vi "Measurement Logic.vi"() -> ()   [LabVIEW 2021, in "Efficiency And Load Regulation_PMIC.lvlib"]
uses:
  Efficiency And Load Regulation_PMIC.lvlib
  Measurement Configuration.ctl
  Measurement Results.ctl
  <vilib>/Plug-In SDKs/Measurements/Measure Call Context/Measure Call Context.lvclass
  <instrlib>/niDCPower/nidcpower.llb/niDCPower Sense.ctl
  <instrlib>/niDCPower/nidcpower.llb/niDCPower Source Mode.ctl
  <instrlib>/niDCPower/nidcpower.llb/niDCPower Wait For Event - Event.ctl
  <instrlib>/niDCPower/nidcpower.llb/niDCPower Output Function.ctl
  <instrlib>/niDCPower/nidcpower.llb/niDCPower Sequence Attribute Type.ctl
  <instrlib>/niDCPower/nidcpower.llb/niDCPower Get Channel Name From String.vi
  <instrlib>/niDCPower/nidcpower.llb/niDCPower Create Advanced Sequence Step With Channels.vi
  <instrlib>/niDCPower/nidcpower.llb/niDCPower Configure Digital Edge Source Trigger With Channels.vi
  <instrlib>/niDCPower/nidcpower.llb/niDCPower Configure Digital Edge Measure Trigger With Channels.vi
panel:
  out "measure call context out":refnum<class "Measure Call Context.lvclass">
  in  "measure call context in":refnum<class "Measure Call Context.lvclass">
  out "measurement results":T1
  in  "measurement configuration":T2={"Mode of operation"=enum."Perform measurement", "DUT setup time"=1.0, "Source delay"=0.005, "Aperture time"=0.005, "Nominal output voltage"=3.3, "Measurement timeout"=10.0, "Source resource name"="", "Source sense"=1009, "Source current limit"=25.0, "Source maximum power"=300.0, "Source start voltage"=5.0, "Source stop voltage"=20.0, "Source voltage sweep points"=10, "Load resource name"="", "Load sense"=1009, "Load voltage limit range"=6.0, "Load sweep type"="Logarithmic", "Load start current"=0.1, "Load stop current"=24.0, "Load current sweep points/points per decade"=10} {"Load sense" items=["Local"=1008, "Remote"=1009]; "Source sense" items=["Local"=1008, "Remote"=1009]}
  out "error out":errorcluster
  in  "error in":errorcluster
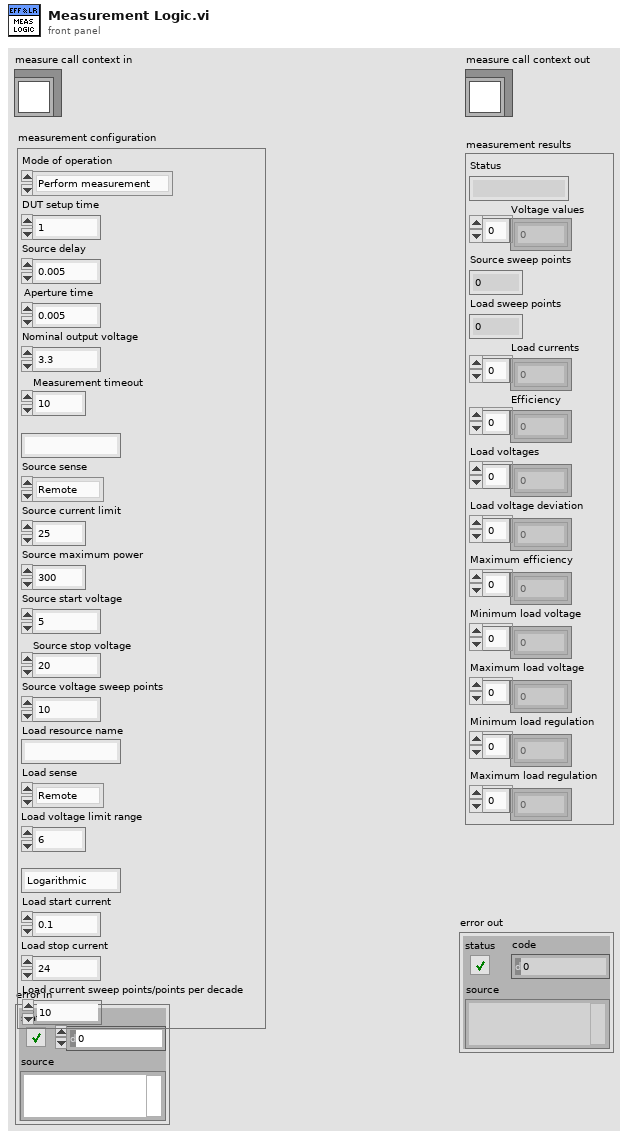
[diagram p1: front panel]
types:
  T1 = typedef "Efficiency And Load Regulation_PMIC.lvlib/Measurement Results.ctl" = cluster{"Status":string, "Voltage values":dbl[], "Source sweep points":i32, "Load sweep points":i32, "Load currents":dbl[], "Efficiency":dbl[], "Load voltages":dbl[], "Load voltage deviation":dbl[], "Maximum efficiency":dbl[], "Minimum load voltage":dbl[], "Maximum load voltage":dbl[], "Minimum load regulation":dbl[], "Maximum load regulation":dbl[]}
  T2 = typedef "Efficiency And Load Regulation_PMIC.lvlib/Measurement Configuration.ctl" = cluster{"Mode of operation":enum32{"Power on the DUT", "Perform measurement", "Power off the DUT"}, "DUT setup time":dbl, "Source delay":dbl, "Aperture time":dbl, "Nominal output voltage":dbl, "Measurement timeout":dbl, "Source resource name":string, "Source sense":i32, "Source current limit":dbl, "Source maximum power":dbl, "Source start voltage":dbl, "Source stop voltage":dbl, "Source voltage sweep points":i32, "Load resource name":string, "Load sense":i32, "Load voltage limit range":dbl, "Load sweep type":string, "Load start current":dbl, "Load stop current":dbl, "Load current sweep points/points per decade":i32}
  T3 = cluster{"Voltage values":dbl[], "Source out":refnum<k15>, "Source channel name":string, "Load out":refnum<k15>, "Load channel name":string, "Current values":dbl[], "Load sweep points":i32, "Source terminal name":string, "Measure terminal name":string, "Measurement Results":T1, "Source sequence name":string}
  T4 = enum32{"Power on the DUT", "Perform measurement", "Power off the DUT"}
  T5 = typedef "niDCPower Wait For Event - Event.ctl" = i32
  T6 = typedef "niDCPower Source Mode.ctl" = i32
  T7 = typedef "niDCPower Sense.ctl" = i32
  T8 = typedef "niDCPower Sequence Attribute Type.ctl" = i32
  T9 = typedef "niDCPower Output Function.ctl" = i32
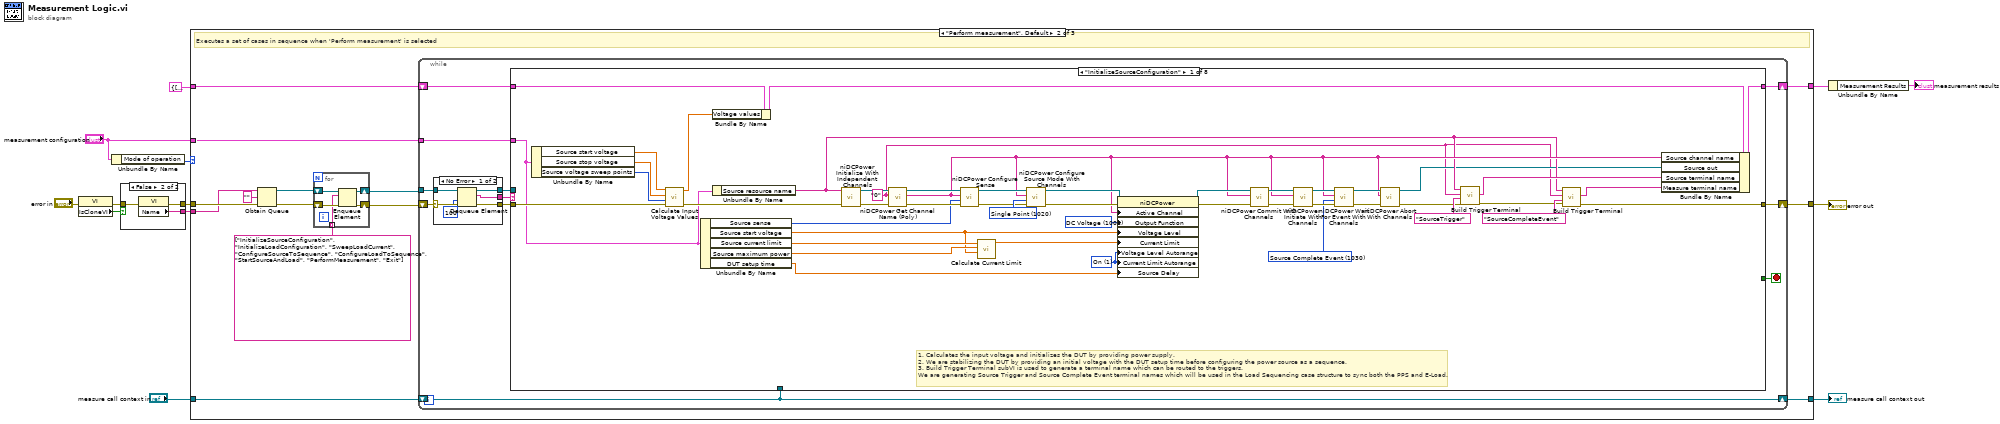
[diagram p0: block diagram]
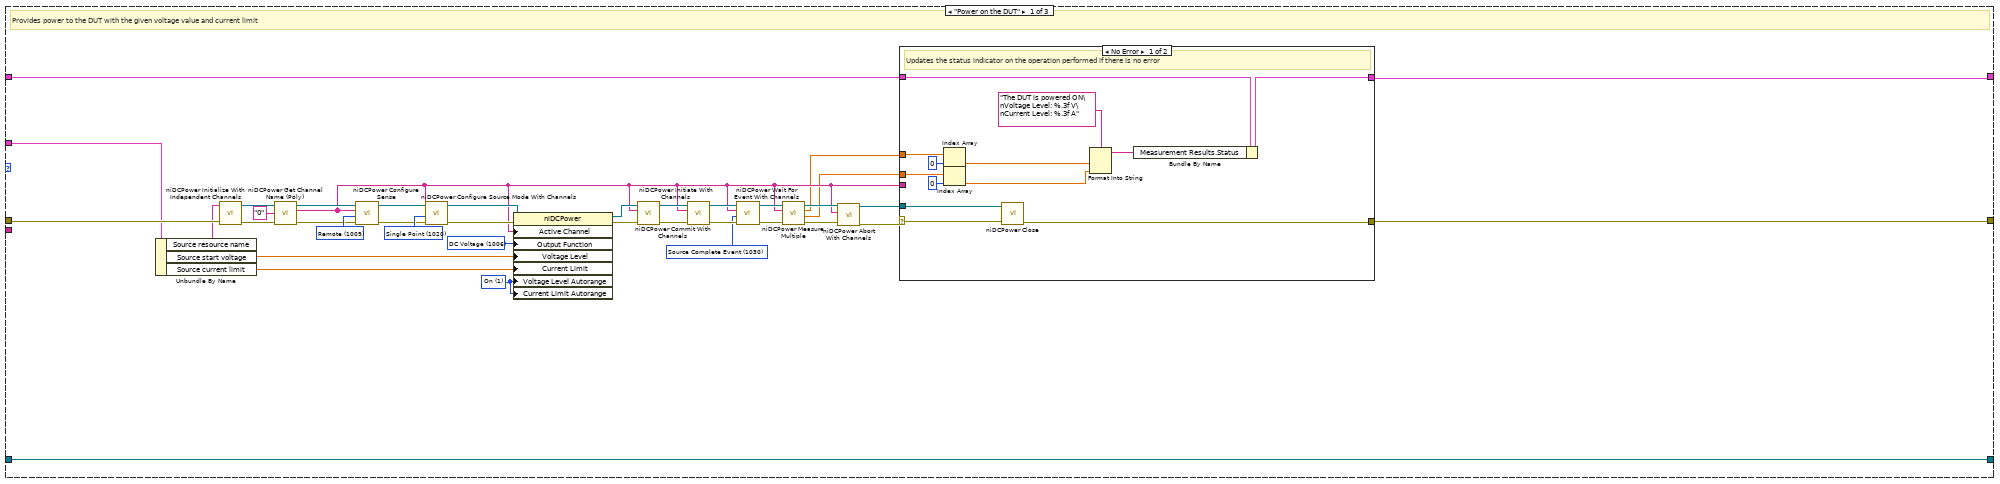
[diagram p2: hidden frame]
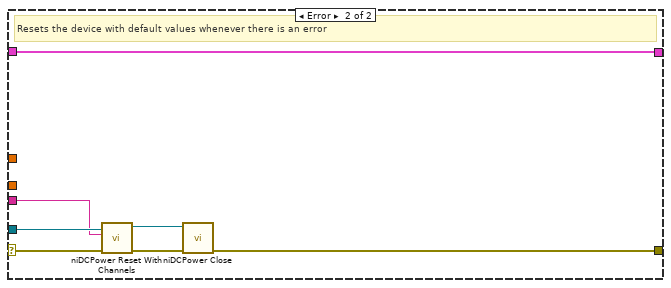
[diagram p3: hidden frame]
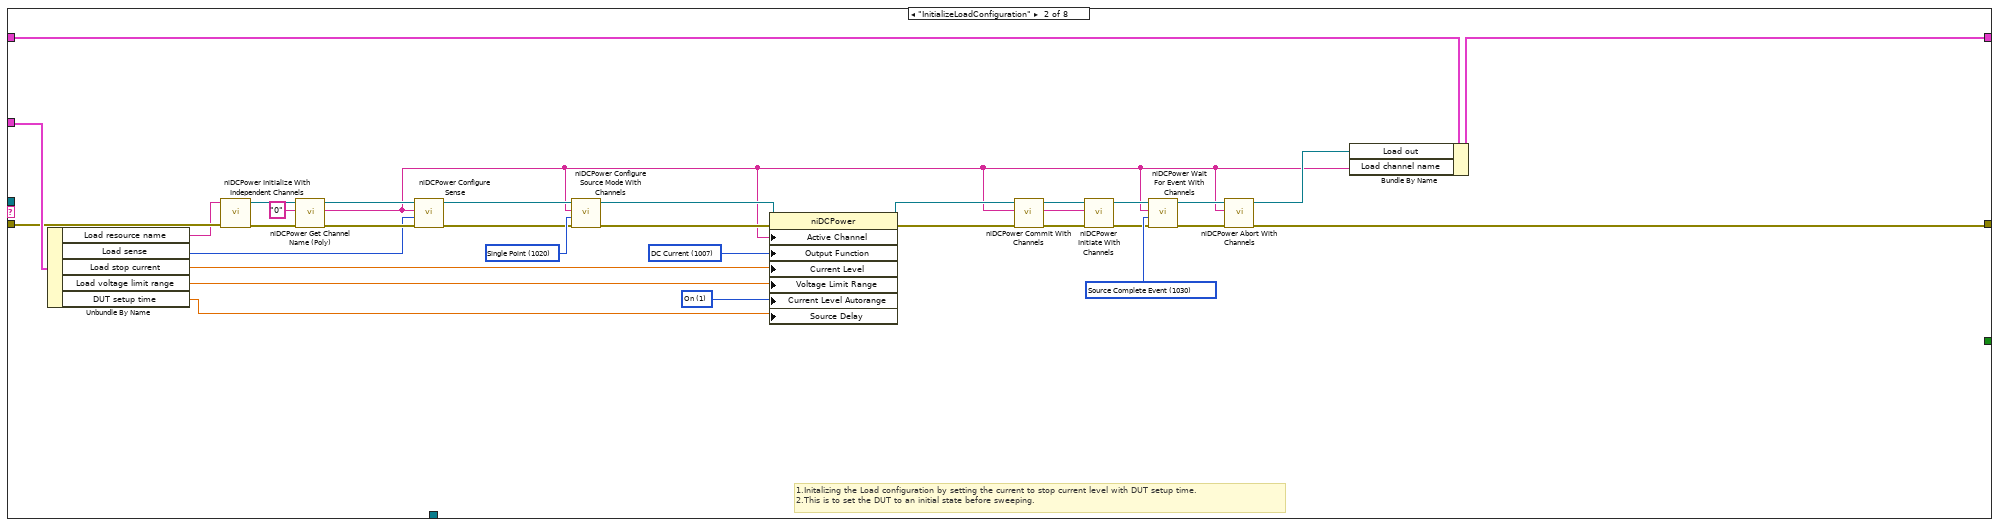
[diagram p4: hidden frame]
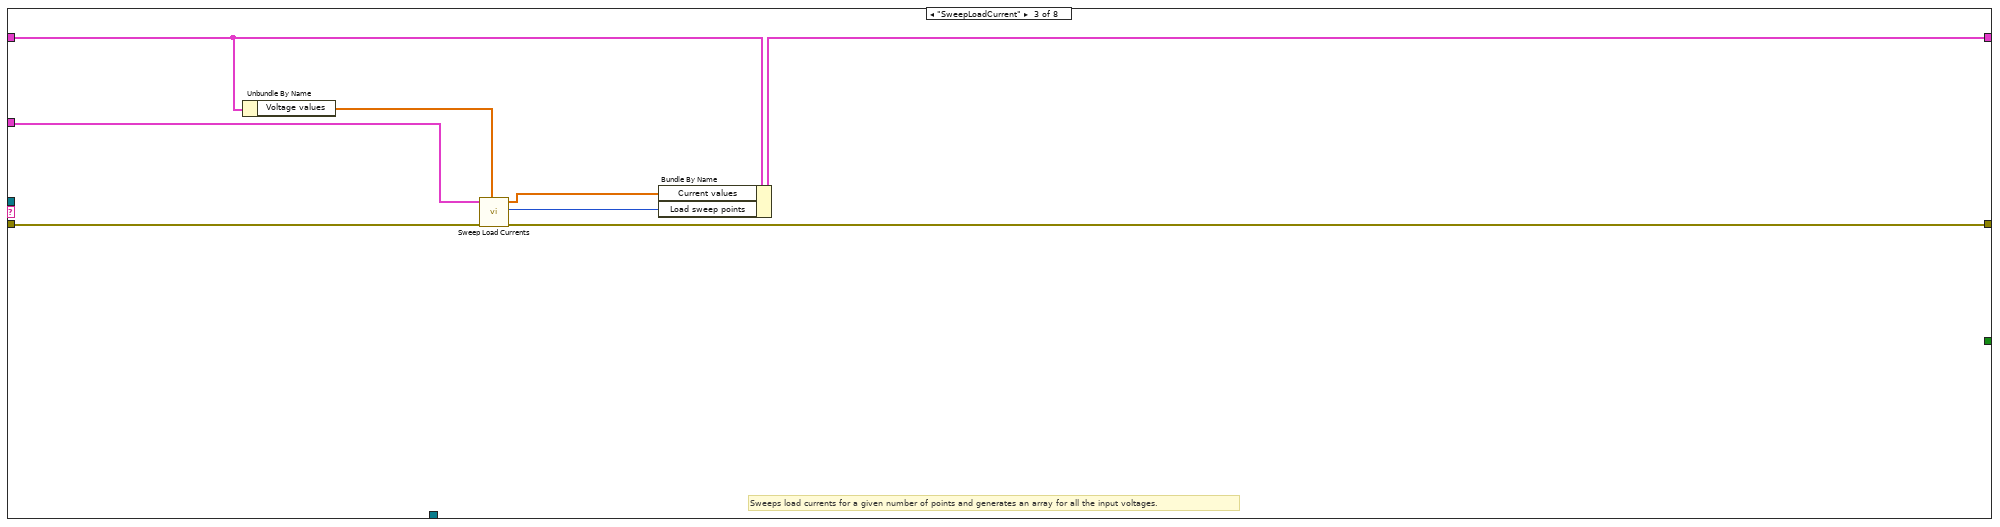
[diagram p5: hidden frame]
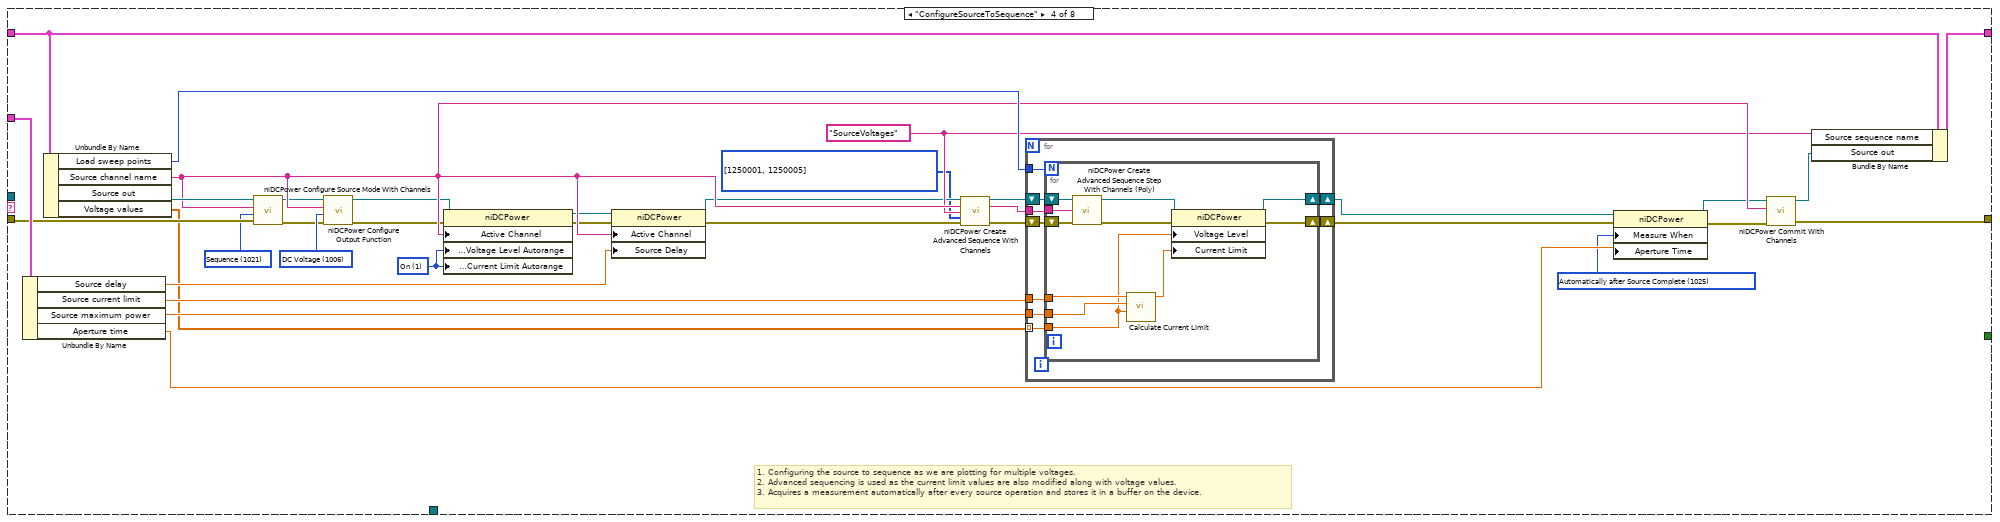
[diagram p6: hidden frame]
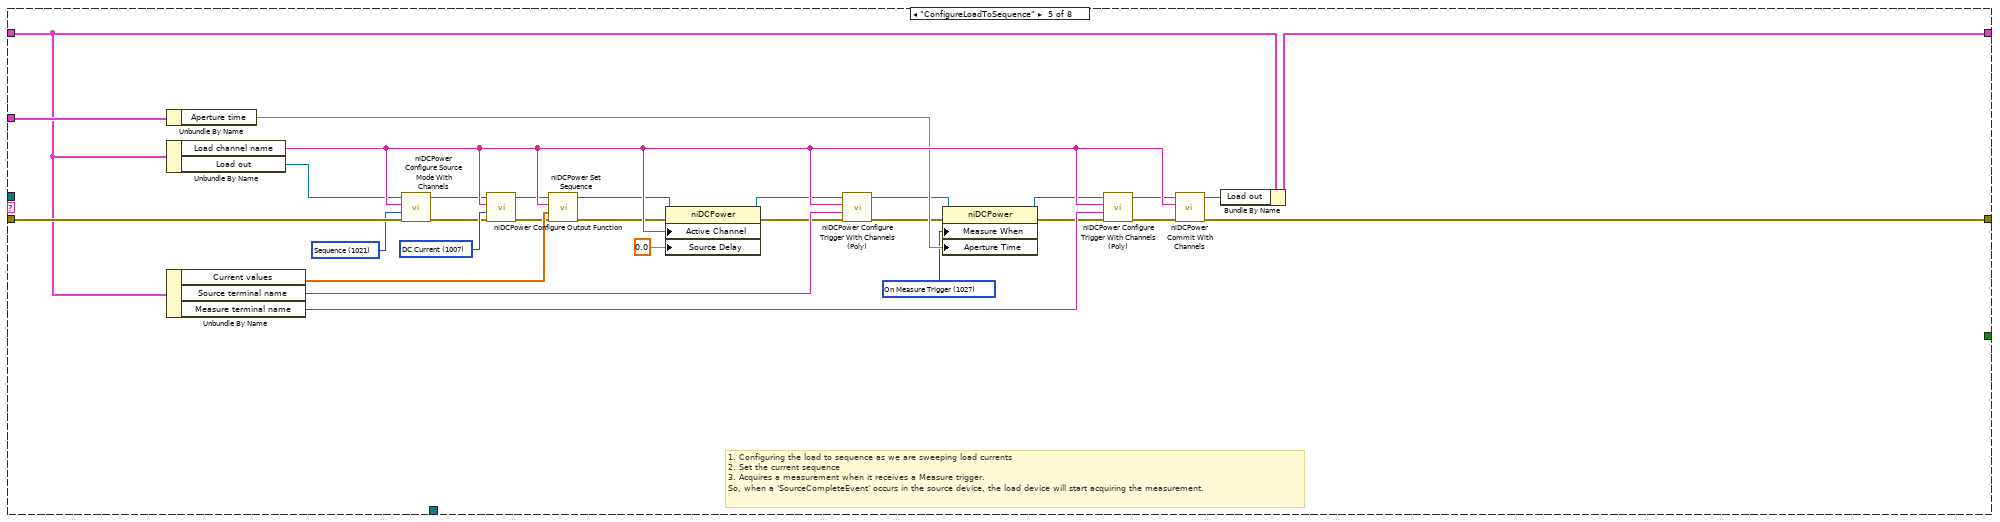
[diagram p7: hidden frame]
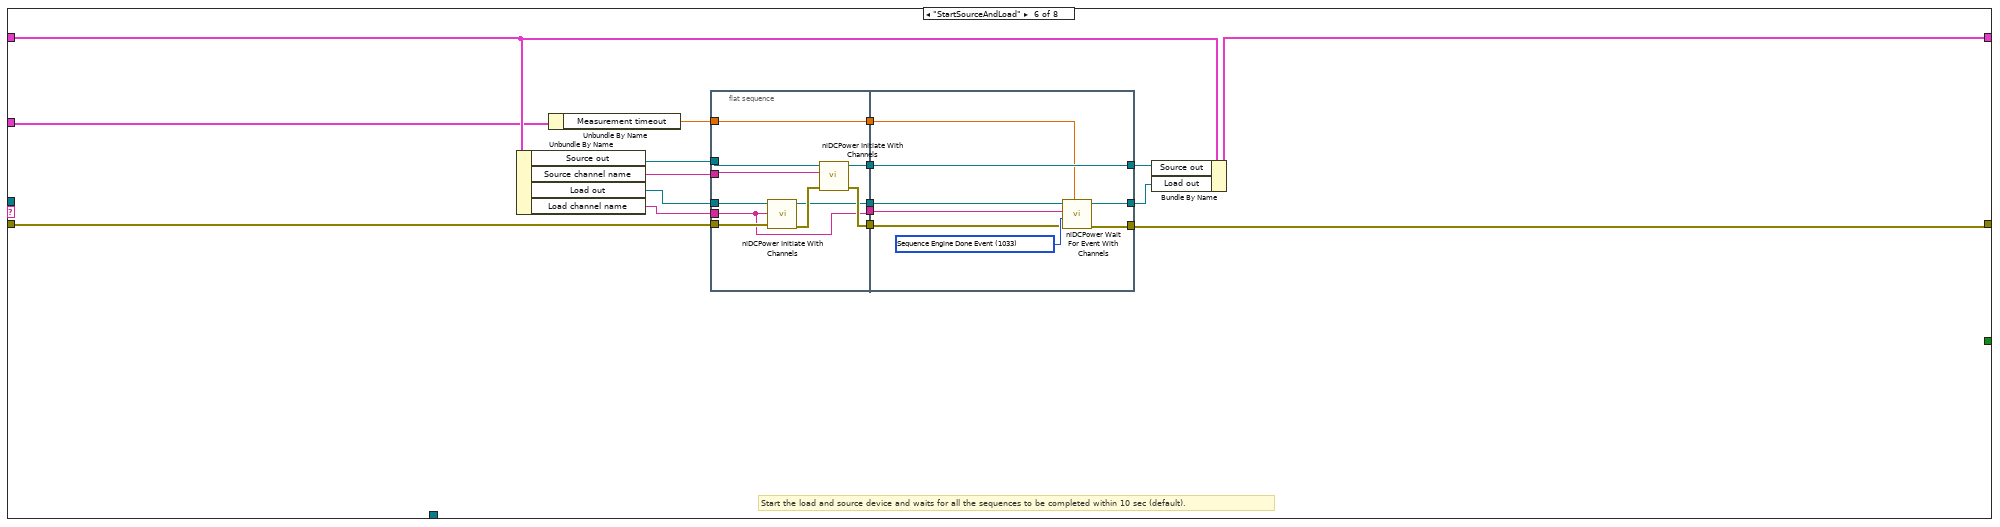
[diagram p8: hidden frame]
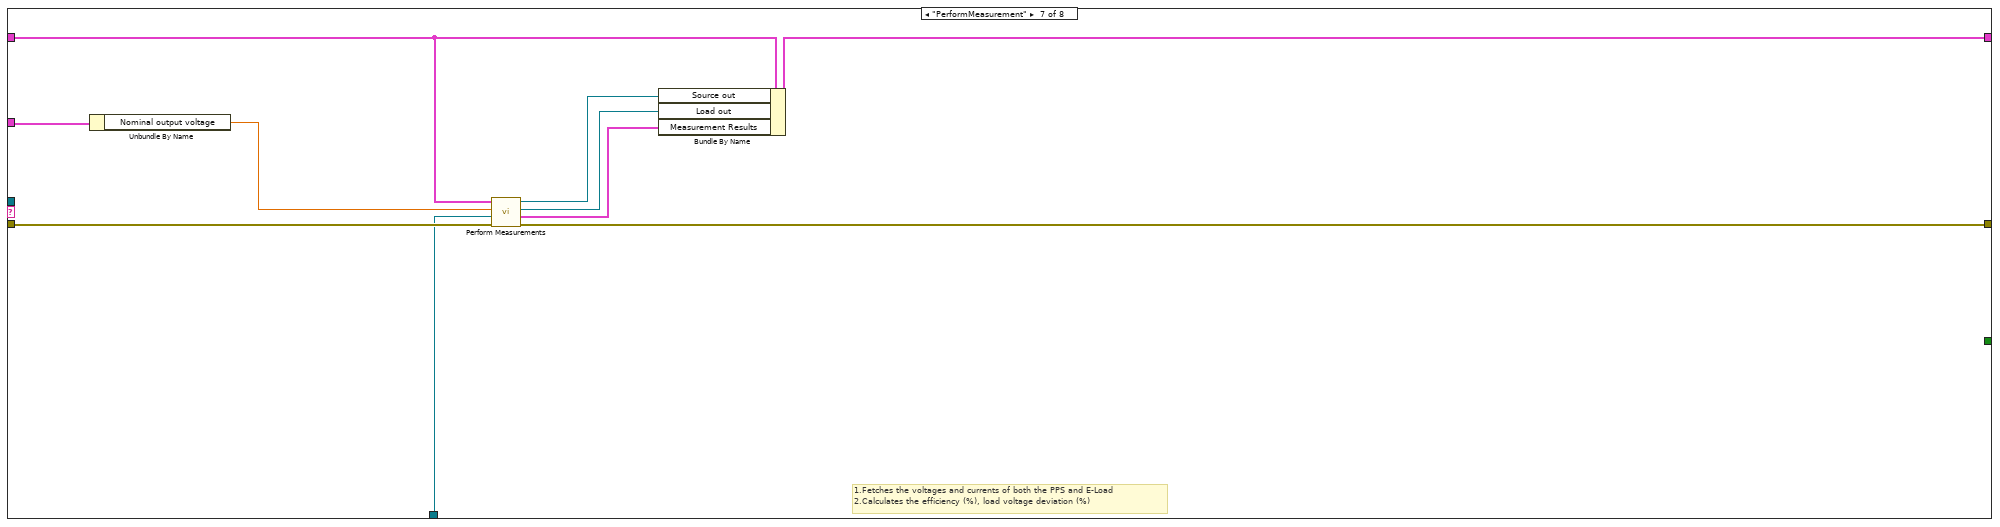
[diagram p9: hidden frame]
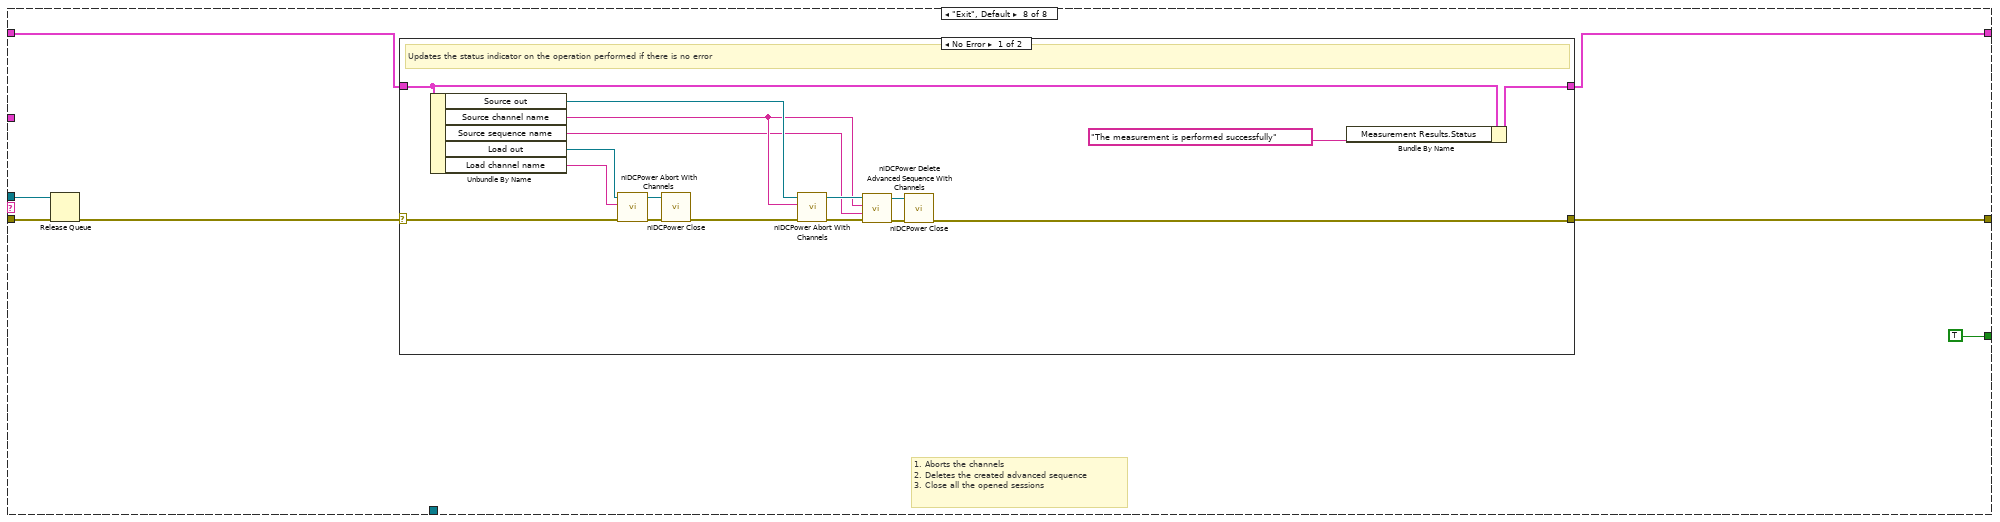
[diagram p10: hidden frame]
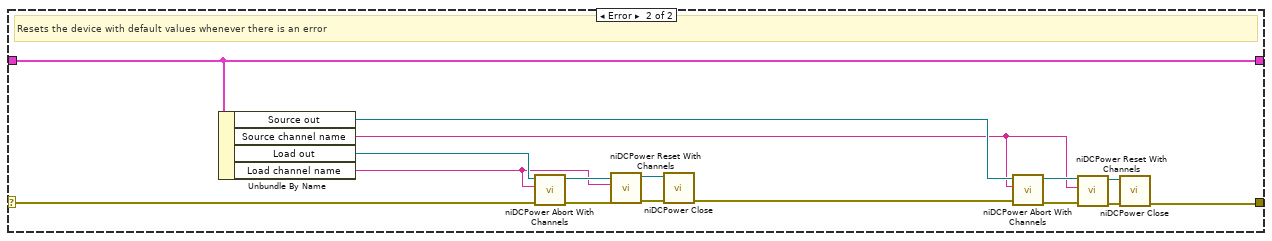
[diagram p11: hidden frame]
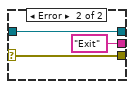
[diagram p12: hidden frame]
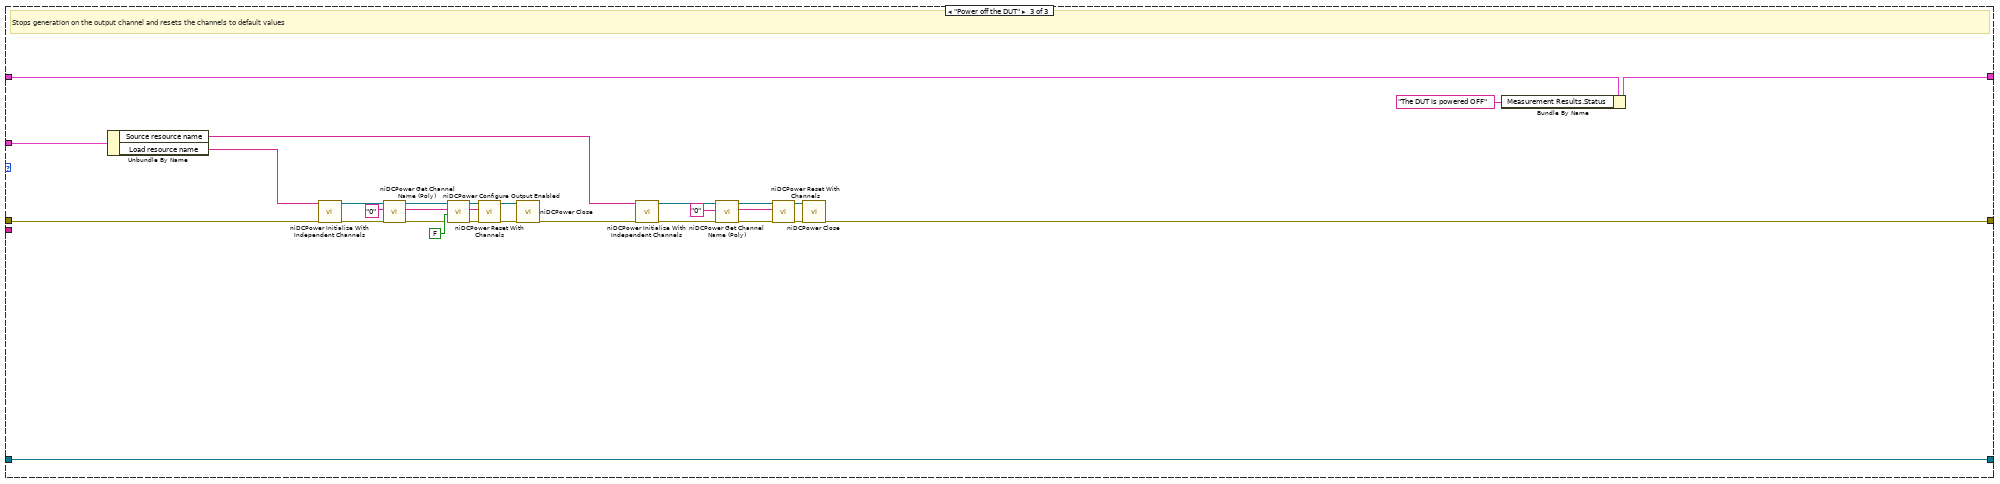
[diagram p13: hidden frame]
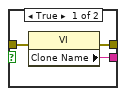
[diagram p14: hidden frame]
diagram:
  n1 = property class="VI"(error in="error in") -> (error out=w12:errorcluster, "IsCloneVI"=w13:bool)  [unwired: 1 in, 1 out]
  n2 = Unbundle By Name("measurement configuration") -> ("Mode of operation"=w5:T4)
  n3 = case shown="False" w13 {
    tunnel: [w16 w19] -> w7
    tunnel: [w15 w18] -> w6
    tunnel: w12 -> [w14 w17]
    frame True {
      n4 = property class="VI"(error in=w14) -> (error out=w16:errorcluster, "Clone Name"=w15:string)  [unwired: 1 in, 1 out]
    }
    frame False {
      n5 = property class="VI"(error in=w17) -> (error out=w19:errorcluster, "Name"=w18:string)  [unwired: 1 in, 1 out]
    }
  }
  n6 = case shown="\"Perform measurement\", Default" w5 {
    tunnel: [w21 w77 w390] -> w1
    tunnel: w7 -> [w37 w87 w389]
    tunnel: w6 -> [_ w86 _]
    tunnel: "measurement configuration" -> [w30 w83 w377]
    tunnel: [w22 w78 w373] -> w2
    tunnel: T3 {"Voltage values"=[], "Source out"="", "Source channel name"="", "Load out"="", "Load channel name"="", "Current values"=[], "Load sweep points"=0, "Source terminal name"="", "Measure terminal name"="", "Measurement Results"={"Status"="", "Voltage values"=[], "Source sweep points"=0, "Load sweep points"=0, "Load currents"=[], "Efficiency"=[], "Load voltages"=[], "Load voltage deviation"=[], "Maximum efficiency"=[], "Minimum load voltage"=[], "Maximum load voltage"=[], "Minimum load regulation"=[], "Maximum load regulation"=[]}, "Source sequence name"=""} -> [w23 w82 w375]
    tunnel: "measure call context in" -> [w20 w80 w376]
    tunnel: [w20 w79 w376] -> w3
    frame "Power on the DUT" {
      w40 = 1 items=["Off", "On"] ("Source:DC Voltage:Voltage Level Autorange")
      w41 = T5 1030 items=["Source Complete Event"=1030, "Measure Complete Event"=1031, "Sequence Iteration Complete Event"=1032, "Sequence Engine Done Event"=1033, "Pulse Complete Event"=1051, "Ready For Pulse Trigger Event"=1052] ("event")
      w52 = T6 1020 items=["Single Point"=1020, "Sequence"=1021] ("source mode")
      w47 = 1006 items=["DC Voltage"=1006, "DC Current"=1007, "Pulse Voltage"=1049, "Pulse Current"=1050] ("Source:Output Function")
      w42 = T7 1009 items=["Local"=1008, "Remote"=1009] ("sense")
      # "Provides power to the DUT with the given voltage value and current limit"
      n7 = Unbundle By Name(w30) -> ("Source resource name"=w34:string, "Source start voltage"=w29:dbl, "Source current limit"=w35:dbl)
      n8 = call <instrlib>:"niDCPower Initialize With Independent Channels.vi"("error in (no error)"=w37, "resource name"=w34) -> ("error out"=w39:errorcluster, "instrument handle out"=w43:refnum<k15>)  [unwired: 8 in]
      n9 = call-poly <instrlib>:"niDCPower Get Channel Name (Poly).vi"("index"="0", "instrument handle"=w43) -> ("name"=w26:string, "instrument handle out"=w38:refnum<k15>)  [unwired: 7 in, 1 out]
      n10 = call <instrlib>:"niDCPower Configure Sense.vi"("error in (no error)"=w39, "sense"=w42, "channel name"=w26, "instrument handle"=w38) -> ("error out"=w50:errorcluster, "instrument handle out"=w48:refnum<k15>)  [unwired: 6 in]
      n11 = call <instrlib>:"niDCPower Configure Source Mode With Channels.vi"("error in (no error)"=w50, "source mode"=w52, "channel name"=w26, "instrument handle"=w48) -> ("error out"=w51:errorcluster, "instrument handle out"=w49:refnum<k15>)  [unwired: 6 in]
      n12 = property class="niDCPower"(reference=w49, error in=w51, "Active Channel"=w26, "Output Function"=w47, "Voltage Level"=w29, "Current Limit"=w35, "Voltage Level Autorange"=w40, "Current Limit Autorange"=w40) -> (reference out=w53:refnum<k15>, error out=w54:errorcluster)
      n13 = call <instrlib>:"niDCPower Commit With Channels.vi"("error in (no error)"=w54, "channel name"=w26, "instrument handle"=w53) -> ("error out"=w56:errorcluster, "instrument handle out"=w55:refnum<k15>)  [unwired: 7 in]
      n14 = call <instrlib>:"niDCPower Initiate With Channels.vi"("error in (no error)"=w56, "channel name"=w26, "instrument handle"=w55) -> ("error out"=w44:errorcluster, "instrument handle out"=w45:refnum<k15>)  [unwired: 7 in]
      n15 = call <instrlib>:"niDCPower Wait For Event With Channels.vi"("error in (no error)"=w44, "event"=w41, "channel name"=w26, "instrument handle"=w45) -> ("error out"=w32:errorcluster, "instrument handle out"=w46:refnum<k15>)  [unwired: 6 in]
      n16 = call <instrlib>:"niDCPower Measure Multiple.vi"("error in (no error)"=w32, "channel name"=w26, "instrument handle"=w46) -> ("error out"=w31:errorcluster, "current measurements"=w24:dbl[], "voltage measurements"=w25:dbl[], "instrument handle out"=w33:refnum<k15>)  [unwired: 5 in]
      n17 = call <instrlib>:"niDCPower Abort With Channels.vi"("error in (no error)"=w31, "channel name"=w26, "instrument handle"=w33) -> ("error out"=w28:errorcluster, "instrument handle out"=w27:refnum<k15>)  [unwired: 7 in]
      n18 = case shown="No Error" w28 {
        selector: w28 -> [w69 w74]
        tunnel: [w68 w73] -> w21
        tunnel: [w67 w70] -> w22
        tunnel: w27 -> [w62 w72]
        tunnel: w26 -> [_ w71]
        tunnel: w25 -> [w61 _]
        tunnel: w24 -> [w60 _]
        tunnel: w23 -> [w59 w70]
        frame No Error {
          # "Updates the status indicator on the operation performed if there is no error"
          n19 = Index Array(array=w61, index=0) -> (element=w58:dbl)
          n20 = Index Array(array=w60, index=0) -> (element=w57:dbl)
          n21 = call <instrlib>:"niDCPower Close.vi"("error in (no error)"=w69, "instrument handle"=w62) -> ("error out"=w68:errorcluster)  [unwired: 9 out]
          n22 = Format Into String(format string="The DUT is powered ON\nVoltage Level: %.3f V\nCurrent Level: %.3f A" ("message"), w58, w57) -> (resulting string=w65:string)  [unwired: 2 in, 1 out]
          n23 = Bundle By Name(cluster=w59, "Measurement Results.Status"=w65) -> (w67:T3)
        }
        frame Error {
          # "Resets the device with default values whenever there is an error"
          n24 = call <instrlib>:"niDCPower Reset With Channels.vi"("error in (no error)"=w74, "channel name"=w71, "instrument handle"=w72) -> ("error out"=w76:errorcluster, "instrument handle out"=w75:refnum<k15>)  [unwired: 7 in]
          n25 = call <instrlib>:"niDCPower Close.vi"("error in (no error)"=w76, "instrument handle"=w75) -> ("error out"=w73:errorcluster)  [unwired: 9 out]
        }
      }
    }
    frame "Perform measurement", Default {
      # "Executes a set of cases in sequence when 'Perform measurement' is selected"
      n26 = Obtain Queue(name (unnamed)=w86, element data type="", error in (no error)=w87) -> (queue out=w89:refnum<queue>, error out=w90:errorcluster)  [unwired: 2 in, 1 out]
      n27 = for {
        shift-right: [w370] -> w84
        shift-left: w89 -> [w372]
        shift-right: [w369] -> w81
        shift-left: w90 -> [w371]
        tunnel: string[] ["InitializeSourceConfiguration", "InitializeLoadConfiguration", "SweepLoadCurrent", "ConfigureSourceToSequence", "ConfigureLoadToSequence", "StartSourceAndLoad", "PerformMeasurement", "Exit"] ("Step sequence") -> [w368] mode=indexing
        n28 = Enqueue Element(queue=w372, element=w368, error in (no error)=w371) -> (queue out=w370:refnum<queue>, error out=w369:errorcluster)  [unwired: 1 in, 1 out]
      }
      n29 = while {
        tunnel: w84 -> [w101]
        tunnel: w83 -> [w97]
        shift-right: [w94] -> w78
        shift-left: w82 -> [w95]
        shift-right: [w93] -> w77
        shift-left: w81 -> [w100]
        shift-right: [w92] -> w79
        shift-left: w80 -> [w92]
        stop <- w91 stop-if-true
        n30 = case shown="No Error" w100 {
          selector: w100 -> [w362 w366]
          tunnel: w101 -> [w364 w365]
          tunnel: [w363 "Exit" ("t")] -> w99
          tunnel: [w361 w366] -> w96
          tunnel: [w359 w365] -> w98
          frame No Error {
            n31 = Dequeue Element(queue=w364, timeout in ms (-1)=100, error in (no error)=w362) -> (queue out=w359:refnum<queue>, element=w363:string, error out=w361:errorcluster)  [unwired: 1 out]
          }
          frame Error {
          }
        }
        n32 = case shown="\"InitializeSourceConfiguration\"" w99 {
          tunnel: w98 -> [_ _ _ _ _ _ _ w320]
          tunnel: w97 -> [w119 w181 w182 w221 w267 w276 w316 _]
          tunnel: w96 -> [w128 w180 w187 w220 w273 w282 w318 w325]
          tunnel: w95 -> [w147 w157 w188 w223 w263 w281 w311 w323]
          tunnel: [w148 w176 w189 w222 w262 w278 w309 w321] -> w94
          tunnel: [w109 w179 w186 w211 w265 w277 w317 w322] -> w93
          tunnel: w92 -> [_ _ _ _ _ _ w310 _]
          tunnel: [_ _ _ _ _ _ _ TRUE] -> w91
          frame "InitializeSourceConfiguration" {
            w104 = "0" ("index")
            w130 = 1 items=["Off", "On"] ("Source:DC Voltage:Voltage Level Autorange")
            w131 = T5 1030 items=["Source Complete Event"=1030, "Measure Complete Event"=1031, "Sequence Iteration Complete Event"=1032, "Sequence Engine Done Event"=1033, "Pulse Complete Event"=1051, "Ready For Pulse Trigger Event"=1052] ("event")
            w142 = T6 1020 items=["Single Point"=1020, "Sequence"=1021] ("source mode")
            w137 = 1006 items=["DC Voltage"=1006, "DC Current"=1007, "Pulse Voltage"=1049, "Pulse Current"=1050] ("Source:Output Function")
            # "1. Calculates the input voltage and initializes the DUT by providing power supply.\n2. We are stabilizing the DUT by providing an initial voltage with the DUT setup time before configuring the power source as a sequence.\n3. Build Trigger Terminal subVI is used to generate a terminal name which can be routed to the triggers. \nWe are generating Source Trigger and Source Complete Event terminal names which will be used in the Load Sequencing case structure to sync both the PPS and E-Load."
            n33 = Unbundle By Name(w119) -> ("Source start voltage"=w125:dbl, "Source stop voltage"=w124:dbl, "Source voltage sweep points"=w123:i32)
            n34 = call "Calculate Input Voltage Values.vi"("error in"=w128, "Points"=w123, "Voltage stop level"=w124, "Voltage start level"=w125) -> ("error out"=w127:errorcluster, "Voltage values"=w126:dbl[])  [unwired: 6 in]
            n35 = Unbundle By Name(w119) -> ("Source sense"=w102:i32, "Source start voltage"=w103:dbl, "Source current limit"=w122:dbl, "Source maximum power"=w121:dbl, "DUT setup time"=w129:dbl)
            n36 = Bundle By Name(cluster=w147, "Voltage values"=w126) -> (w118:T3)
            n37 = Unbundle By Name(w119) -> ("Source resource name"=w106:string)
            n38 = call <instrlib>:"niDCPower Initialize With Independent Channels.vi"("error in (no error)"=w127, "resource name"=w106) -> ("error out"=w115:errorcluster, "instrument handle out"=w132:refnum<k15>)  [unwired: 8 in]
            n39 = call-poly <instrlib>:"niDCPower Get Channel Name (Poly).vi"("error in (no error)"=w115, "index"=w104, "instrument handle"=w132) -> ("error out"=w114:errorcluster, "name"=w116:string, "instrument handle out"=w117:refnum<k15>)  [unwired: 6 in]
            n40 = call <instrlib>:"niDCPower Configure Sense.vi"("error in (no error)"=w114, "sense"=w102, "channel name"=w116, "instrument handle"=w117) -> ("error out"=w140:errorcluster, "instrument handle out"=w138:refnum<k15>)  [unwired: 6 in]
            n41 = call "Calculate Current Limit.vi"("Voltage value"=w103, "Maximum power"=w121, "Current limit in"=w122) -> ("Current limit out"=w120:dbl)  [unwired: 8 in]
            n42 = call <instrlib>:"niDCPower Configure Source Mode With Channels.vi"("error in (no error)"=w140, "source mode"=w142, "channel name"=w116, "instrument handle"=w138) -> ("error out"=w141:errorcluster, "instrument handle out"=w139:refnum<k15>)  [unwired: 6 in]
            n43 = property class="niDCPower"(reference=w139, error in=w141, "Active Channel"=w116, "Output Function"=w137, "Voltage Level"=w103, "Current Limit"=w120, "Voltage Level Autorange"=w130, "Current Limit Autorange"=w130, "Source Delay"=w129) -> (reference out=w143:refnum<k15>, error out=w144:errorcluster)
            n44 = call <instrlib>:"niDCPower Commit With Channels.vi"("error in (no error)"=w144, "channel name"=w116, "instrument handle"=w143) -> ("error out"=w146:errorcluster, "instrument handle out"=w145:refnum<k15>)  [unwired: 7 in]
            n45 = call <instrlib>:"niDCPower Initiate With Channels.vi"("error in (no error)"=w146, "channel name"=w116, "instrument handle"=w145) -> ("error out"=w133:errorcluster, "instrument handle out"=w134:refnum<k15>)  [unwired: 7 in]
            n46 = call <instrlib>:"niDCPower Wait For Event With Channels.vi"("error in (no error)"=w133, "event"=w131, "channel name"=w116, "instrument handle"=w134) -> ("error out"=w136:errorcluster, "instrument handle out"=w135:refnum<k15>)  [unwired: 6 in]
            n47 = call <instrlib>:"niDCPower Abort With Channels.vi"("error in (no error)"=w136, "channel name"=w116, "instrument handle"=w135) -> ("error out"=w111:errorcluster, "instrument handle out"=w105:refnum<k15>)  [unwired: 7 in]
            n48 = call "Build Trigger Terminal.vi"("error in (no error)"=w111, "Trigger/Event Name"="SourceTrigger", "Channel Name"=w104, "Resource Name"=w106) -> ("error out"=w110:errorcluster, "Terminal Name"=w108:string)  [unwired: 6 in]
            n49 = call "Build Trigger Terminal.vi"("error in (no error)"=w110, "Trigger/Event Name"="SourceCompleteEvent", "Channel Name"=w104, "Resource Name"=w106) -> ("error out"=w109:errorcluster, "Terminal Name"=w107:string)  [unwired: 6 in]
            n50 = Bundle By Name(cluster=w118, "Source channel name"=w116, "Source out"=w105, "Source terminal name"=w108, "Measure terminal name"=w107) -> (w148:T3)
          }
          frame "InitializeLoadConfiguration" {
            w171 = T6 1020 items=["Single Point"=1020, "Sequence"=1021] ("source mode")
            w164 = T5 1030 items=["Source Complete Event"=1030, "Measure Complete Event"=1031, "Sequence Iteration Complete Event"=1032, "Sequence Engine Done Event"=1033, "Pulse Complete Event"=1051, "Ready For Pulse Trigger Event"=1052] ("event")
            w159 = 1 items=["Off", "On"] ("Source:DC Current:Current Level Autorange")
            w160 = 1007 items=["DC Voltage"=1006, "DC Current"=1007, "Pulse Voltage"=1049, "Pulse Current"=1050] ("Source:Output Function")
            # "1.Initalizing the Load configuration by setting the current to stop current level with DUT setup time.\n2.This is to set the DUT to an initial state before sweeping."
            n51 = Unbundle By Name(w181) -> ("Load resource name"=w150:string, "Load sense"=w149:i32, "Load stop current"=w151:dbl, "Load voltage limit range"=w178:dbl, "DUT setup time"=w158:dbl)
            n52 = call <instrlib>:"niDCPower Initialize With Independent Channels.vi"("error in (no error)"=w180, "resource name"=w150) -> ("error out"=w153:errorcluster, "instrument handle out"=w161:refnum<k15>)  [unwired: 8 in]
            n53 = call-poly <instrlib>:"niDCPower Get Channel Name (Poly).vi"("error in (no error)"=w153, "index"="0", "instrument handle"=w161) -> ("error out"=w152:errorcluster, "name"=w154:string, "instrument handle out"=w156:refnum<k15>)  [unwired: 6 in]
            n54 = call <instrlib>:"niDCPower Configure Sense.vi"("error in (no error)"=w152, "sense"=w149, "channel name"=w154, "instrument handle"=w156) -> ("error out"=w168:errorcluster, "instrument handle out"=w167:refnum<k15>)  [unwired: 6 in]
            n55 = call <instrlib>:"niDCPower Configure Source Mode With Channels.vi"("error in (no error)"=w168, "source mode"=w171, "channel name"=w154, "instrument handle"=w167) -> ("error out"=w170:errorcluster, "instrument handle out"=w169:refnum<k15>)  [unwired: 6 in]
            n56 = property class="niDCPower"(reference=w169, error in=w170, "Active Channel"=w154, "Output Function"=w160, "Current Level"=w151, "Voltage Limit Range"=w178, "Current Level Autorange"=w159, "Source Delay"=w158) -> (reference out=w172:refnum<k15>, error out=w173:errorcluster)
            n57 = call <instrlib>:"niDCPower Commit With Channels.vi"("error in (no error)"=w173, "channel name"=w154, "instrument handle"=w172) -> ("error out"=w174:errorcluster, "instrument handle out"=w175:refnum<k15>)  [unwired: 7 in]
            n58 = call <instrlib>:"niDCPower Initiate With Channels.vi"("error in (no error)"=w174, "channel name"=w154, "instrument handle"=w175) -> ("error out"=w162:errorcluster, "instrument handle out"=w163:refnum<k15>)  [unwired: 7 in]
            n59 = call <instrlib>:"niDCPower Wait For Event With Channels.vi"("error in (no error)"=w162, "event"=w164, "channel name"=w154, "instrument handle"=w163) -> ("error out"=w166:errorcluster, "instrument handle out"=w165:refnum<k15>)  [unwired: 6 in]
            n60 = call <instrlib>:"niDCPower Abort With Channels.vi"("error in (no error)"=w166, "channel name"=w154, "instrument handle"=w165) -> ("error out"=w179:errorcluster, "instrument handle out"=w177:refnum<k15>)  [unwired: 7 in]
            n61 = Bundle By Name(cluster=w157, "Load out"=w177, "Load channel name"=w154) -> (w176:T3)
          }
          frame "SweepLoadCurrent" {
            # "Sweeps load currents for a given number of points and generates an array for all the input voltages."
            n62 = Unbundle By Name(w188) -> ("Voltage values"=w183:dbl[])
            n63 = call "Sweep Load Currents.vi"("Voltage values"=w183, "error in"=w187, "Measurement Configuration"=w182) -> ("error out"=w186:errorcluster, "Load sweep points"=w185:i32, "Current values"=w184:dbl[])  [unwired: 6 in]
            n64 = Bundle By Name(cluster=w188, "Current values"=w184, "Load sweep points"=w185) -> (w189:T3)
          }
          frame "ConfigureSourceToSequence" {
            w193 = 1025 items=["Automatically after Source Complete"=1025, "On Demand"=1026, "On Measure Trigger"=1027] ("Measurement:Advanced:Measure When")
            w201 = 1 items=["Off", "On"] ("DC Voltage:Voltage Level Autorange")
            w200 = T8[] [1250001, 1250005] items=["Source -> Output Function"=1150008, "Source -> Output Enabled"=1250006, "Source -> Output Resistance"=1150061, "Source -> Transient Response"=1150062, "Source -> Custom Transient Response -> Voltage Gain Bandwidth"=1150067, "Source -> Custom Transient Response -> Voltage Compensation Frequency"=1150068, "Source -> Custom Transient Response -> Voltage Pole-Zero Ratio"=1150069, "Source -> Custom Transient Response -> Current Gain Bandwidth"=1150070, "Source -> Custom Transient Response -> Current Compensation Frequency"=1150071, "Source -> Custom Transient Response -> Current Pole-Zero Ratio"=1150072, "Source -> DC Voltage -> Voltage Level"=1250001, "Source -> DC Voltage -> Voltage Level Range"=1150005, "Source -> DC Voltage -> Current Limit"=1250005, "Source -> DC Voltage -> Current Limit High"=1150187, "Source -> DC Voltage -> Current Limit Low"=1150188, "Source -> DC Voltage -> Current Limit Range"=1150004, "Source -> DC Current -> Current Level"=1150009, "Source -> DC Current -> Current Level Range"=1150011, "Source -> DC Current -> Voltage Limit"=1150010, "Source -> DC Current -> Voltage Limit High"=1150185, "Source -> DC Current -> Voltage Limit Low"=1150186, "Source -> DC Current -> Voltage Limit Range"=1150012, "Source -> Pulse Voltage -> Pulse Voltage Level"=1150080, "Source -> Pulse Voltage -> Pulse Bias Voltage Level"=1150082, "Source -> Pulse Voltage -> Pulse Voltage Level Range"=1150084, "Source -> Pulse Voltage -> Pulse Current Limit"=1150081, "Source -> Pulse Voltage -> Pulse Current Limit High"=1150193, "Source -> Pulse Voltage -> Pulse Current Limit Low"=1150194, "Source -> Pulse Voltage -> Pulse Bias Current Limit"=1150083, "Source -> Pulse Voltage -> Pulse Bias Current Limit High"=1150195, "Source -> Pulse Voltage -> Pulse Bias Current Limit Low"=1150196, "Source -> Pulse Voltage -> Pulse Current Limit Range"=1150085, "Source -> Pulse Current -> Pulse Current Level"=1150086, "Source -> Pulse Current -> Pulse Bias Current Level"=1150088, "Source -> Pulse Current -> Pulse Current Level Range"=1150090, "Source -> Pulse Current -> Pulse Voltage Limit"=1150087, "Source -> Pulse Current -> Pulse Voltage Limit High"=1150189, "Source -> Pulse Current -> Pulse Voltage Limit Low"=1150190, "Source -> Pulse Current -> Pulse Bias Voltage Limit"=1150089, "Source -> Pulse Current -> Pulse Bias Voltage Limit High"=1150191, "Source -> Pulse Current -> Pulse Bias Voltage Limit Low"=1150192, "Source -> Pulse Current -> Pulse Voltage Limit Range"=1150091, "Source -> Advanced -> Source Delay"=1150051, "Source -> Advanced -> Pulse Bias Delay"=1150092, "Source -> Advanced -> Pulse On Time"=1150093, "Source -> Advanced -> Pulse Off Time"=1150094, "Source -> Advanced -> OVP Enabled"=1250002, "Source -> Advanced -> OVP Limit"=1250003, "Source -> Advanced -> Compliance Limit Symmetry"=1150184, "Source -> Advanced -> Sequence Step Delta Time"=1150198, "Measurement -> Sense"=1150013, "Measurement -> Aperture Time"=1150058, "Measurement -> Measure Record Length"=1150063, "Measurement -> Advanced -> DC Noise Rejection"=1150066, "Measurement -> Autorange"=1150244, "Measurement -> Advanced -> Autorange Behavior"=1150245, "Measurement -> Advanced -> Autorange Aperture Time Mode"=1150246, "Measurement -> Advanced -> Autorange Minimum Aperture Time"=1150247, "Measurement -> Advanced -> Autorange Minimum Aperture Time Units"=1150248, "Measurement -> Advanced -> Autorange Minimum Current Range"=1150255, "Measurement -> Advanced -> Autorange Minimum Voltage Range"=1150256, "Measurement -> Advanced -> Autorange Threshold Mode"=1150257, "Measurement -> Advanced -> Autorange Maximum Delay After Range Change"=1150322, "LCR -> Instrument Mode"=1150208, "LCR -> LCR Stimulus Function"=1150209, "LCR -> LCR Frequency"=1150210, "LCR -> LCR Voltage Amplitude"=1150211, "LCR -> LCR Current Amplitude"=1150212, "LCR -> LCR DC Bias Source"=1150213, "LCR -> LCR DC Bias Voltage Level"=1150214, "LCR -> LCR DC Bias Current Level"=1150215, "LCR -> LCR Impedance Autorange"=1150216, "LCR -> LCR Impedance Range"=1150217, "LCR -> LCR Measurement Time"=1150218, "LCR -> LCR Custom Measurement Time"=1150258, "LCR -> LCR Source Delay Mode"=1150315, "LCR -> Compensation -> Open -> Enabled"=1150220, "LCR -> Compensation -> Open -> Conductance"=1150261, "LCR -> Compensation -> Open -> Susceptance"=1150262, "LCR -> Compensation -> Short -> Enabled"=1150221, "LCR -> Compensation -> Short -> Resistance"=1150263, "LCR -> Compensation -> Short -> Reactance"=1150264, "LCR -> Compensation -> Load -> Enabled"=1150222, "LCR -> Compensation -> Load -> Measured Resistance"=1150268, "LCR -> Compensation -> Load -> Measured Reactance"=1150269, "LCR -> Compensation -> Load -> Actual Resistance"=1150270, "LCR -> Compensation -> Load -> Actual Reactance"=1150271] ("advanced sequence properties")
            w210 = "SourceVoltages" ("sequence name")
            w197 = T9 1006 items=["DC Voltage"=1006, "DC Current"=1007, "Pulse Voltage"=1049, "Pulse Current"=1050] ("output function")
            w196 = T6 1021 items=["Single Point"=1020, "Sequence"=1021] ("source mode")
            # "1. Configuring the source to sequence as we are plotting for multiple voltages.\n2. Advanced sequencing is used as the current limit values are also modified along with voltage values.\n3. Acquires a measurement automatically after every source operation and stores it in a buffer on the device."
            n65 = Unbundle By Name(w221) -> ("Source delay"=w219:dbl, "Source current limit"=w218:dbl, "Source maximum power"=w217:dbl, "Aperture time"=w216:dbl)
            n66 = Unbundle By Name(w223) -> ("Load sweep points"=w214:i32, "Source channel name"=w213:string, "Source out"=w215:refnum<k15>, "Voltage values"=w212:dbl[])
            n67 = call <instrlib>:"niDCPower Configure Source Mode With Channels.vi"("error in (no error)"=w220, "source mode"=w196, "channel name"=w213, "instrument handle"=w215) -> ("error out"=w194:errorcluster, "instrument handle out"=w195:refnum<k15>)  [unwired: 6 in]
            n68 = call <instrlib>:"niDCPower Configure Output Function.vi"("error in (no error)"=w194, "output function"=w197, "channel name"=w213, "instrument handle"=w195) -> ("error out"=w205:errorcluster, "instrument handle out"=w204:refnum<k15>)  [unwired: 6 out]
            n69 = property class="niDCPower"(reference=w204, error in=w205, "Active Channel"=w213, "Source:DC Voltage:Voltage Level Autorange"=w201, "Source:DC Voltage:Current Limit Autorange"=w201) -> (reference out=w202:refnum<k15>, error out=w203:errorcluster)
            n70 = property class="niDCPower"(reference=w202, error in=w203, "Active Channel"=w213, "Source Delay"=w219) -> (reference out=w208:refnum<k15>, error out=w209:errorcluster)
            n71 = call <instrlib>:"niDCPower Create Advanced Sequence With Channels.vi"("instrument handle"=w208, "channel name"=w213, "sequence name"=w210, "advanced sequence properties"=w200, "error in (no error)"=w209) -> ("instrument handle out"=w198:refnum<k15>, "error out"=w199:errorcluster)  [unwired: 9 in]
            n72 = for {
              tunnel: w217 -> [w228]
              tunnel: w218 -> [w227]
              tunnel: w212 -> [w226] mode=indexing
              shift-right: [w230] -> w206
              shift-left: w198 -> [w232]
              shift-right: [w229] -> w207
              shift-left: w199 -> [w231]
              tunnel: w214 -> [w225]
              tunnel: w213 -> [w224]
              n73 = for {
                N: w225 -> [_]
                shift-right: [w240] -> w229
                shift-left: w231 -> [w243]
                shift-right: [w239] -> w230
                shift-left: w232 -> [w238]
                tunnel: w228 -> [w235]
                tunnel: w226 -> [w233]
                tunnel: w227 -> [w236]
                tunnel: w224 -> [w237]
                n74 = call-poly <instrlib>:"niDCPower Create Advanced Sequence Step With Channels (Poly).vi"("error in (no error)"=w243, "channel name"=w237, "instrument handle"=w238) -> ("error out"=w241:errorcluster, "instrument handle out"=w242:refnum<k15>)  [unwired: 7 in]
                n75 = call "Calculate Current Limit.vi"("Voltage value"=w233, "Maximum power"=w235, "Current limit in"=w236) -> ("Current limit out"=w234:dbl)  [unwired: 8 in]
                n76 = property class="niDCPower"(reference=w242, error in=w241, "Voltage Level"=w233, "Current Limit"=w234) -> (reference out=w239:refnum<k15>, error out=w240:errorcluster)
              }
            }
            n77 = property class="niDCPower"(reference=w206, error in=w207, "Measure When"=w193, "Aperture Time"=w216) -> (reference out=w191:refnum<k15>, error out=w192:errorcluster)
            n78 = call <instrlib>:"niDCPower Commit With Channels.vi"("error in (no error)"=w192, "channel name"=w213, "instrument handle"=w191) -> ("error out"=w211:errorcluster, "instrument handle out"=w190:refnum<k15>)  [unwired: 7 in]
            n79 = Bundle By Name(cluster=w223, "Source sequence name"=w210, "Source out"=w190) -> (w222:T3)
          }
          frame "ConfigureLoadToSequence" {
            w251 = T9 1007 items=["DC Voltage"=1006, "DC Current"=1007, "Pulse Voltage"=1049, "Pulse Current"=1050] ("output function")
            w250 = 1027 items=["Automatically after Source Complete"=1025, "On Demand"=1026, "On Measure Trigger"=1027] ("Measurement:Advanced:Measure When")
            w249 = T6 1021 items=["Single Point"=1020, "Sequence"=1021] ("source mode")
            # "1. Configuring the load to sequence as we are sweeping load currents\n2. Set the current sequence\n3. Acquires a measurement when it receives a Measure trigger. \nSo, when a 'SourceCompleteEvent' occurs in the source device, the load device will start acquiring the measurement."
            n80 = Unbundle By Name(w267) -> ("Aperture time"=w266:dbl)
            n81 = Unbundle By Name(w263) -> ("Load channel name"=w272:string, "Load out"=w271:refnum<k15>)
            n82 = Unbundle By Name(w263) -> ("Current values"=w270:dbl[], "Source terminal name"=w269:string, "Measure terminal name"=w268:string)
            n83 = call <instrlib>:"niDCPower Configure Source Mode With Channels.vi"("error in (no error)"=w273, "source mode"=w249, "channel name"=w272, "instrument handle"=w271) -> ("error out"=w247:errorcluster, "instrument handle out"=w248:refnum<k15>)  [unwired: 6 in]
            n84 = call <instrlib>:"niDCPower Configure Output Function.vi"("error in (no error)"=w247, "output function"=w251, "channel name"=w272, "instrument handle"=w248) -> ("error out"=w260:errorcluster, "instrument handle out"=w259:refnum<k15>)  [unwired: 6 out]
            n85 = call <instrlib>:"niDCPower Set Sequence.vi"("error in (no error)"=w260, "values"=w270, "channel name"=w272, "instrument handle"=w259) -> ("error out"=w255:errorcluster, "instrument handle out"=w254:refnum<k15>)  [unwired: 1 in, 5 out]
            n86 = property class="niDCPower"(reference=w254, error in=w255, "Active Channel"=w272, "Source Delay"=0.0 ("Source:Advanced:Source Delay")) -> (reference out=w252:refnum<k15>, error out=w253:errorcluster)
            n87 = call-poly <instrlib>:"niDCPower Configure Trigger With Channels (Poly).vi"("error in (no error)"=w253, "input terminal"=w269, "channel name"=w272, "instrument handle"=w252) -> ("error out"=w244:errorcluster, "instrument handle out"=w261:refnum<k15>)  [unwired: 6 in]
            n88 = property class="niDCPower"(reference=w261, error in=w244, "Measure When"=w250, "Aperture Time"=w266) -> (reference out=w246:refnum<k15>, error out=w245:errorcluster)
            n89 = call-poly <instrlib>:"niDCPower Configure Trigger With Channels (Poly).vi"("error in (no error)"=w245, "input terminal"=w268, "channel name"=w272, "instrument handle"=w246) -> ("error out"=w256:errorcluster, "instrument handle out"=w257:refnum<k15>)  [unwired: 6 in]
            n90 = call <instrlib>:"niDCPower Commit With Channels.vi"("error in (no error)"=w256, "channel name"=w272, "instrument handle"=w257) -> ("error out"=w265:errorcluster, "instrument handle out"=w264:refnum<k15>)  [unwired: 7 in]
            n91 = Bundle By Name(cluster=w263, "Load out"=w264) -> (w262:T3)
          }
          frame "StartSourceAndLoad" {
            # "Start the load and source device and waits for all the sequences to be completed within 10 sec (default)."
            n92 = Unbundle By Name(w281) -> ("Source out"=w286:refnum<k15>, "Source channel name"=w283:string, "Load out"=w285:refnum<k15>, "Load channel name"=w284:string)
            n93 = Unbundle By Name(w276) -> ("Measurement timeout"=w274:dbl)
            n94 = flat-sequence {
              tunnel: [w299] -> w290
              tunnel: [w298] -> w289
              tunnel: [w297] -> w288
              tunnel: w282 -> [w296]
              tunnel: w285 -> [w295]
              tunnel: w286 -> [w294]
              tunnel: w283 -> [w293]
              tunnel: [w292] -> w287
              tunnel: w284 -> [w292]
              tunnel: [w291] -> w275
              tunnel: w274 -> [w291]
              tunnel: w290 -> [w308]
              tunnel: w289 -> [w306]
              tunnel: w288 -> [w303]
              tunnel: [w308] -> w280
              tunnel: [w304] -> w277
              tunnel: [w305] -> w279
              tunnel: w287 -> [w302]
              tunnel: w275 -> [w301]
              frame #0 {
                n95 = call <instrlib>:"niDCPower Initiate With Channels.vi"("error in (no error)"=w296, "channel name"=w292, "instrument handle"=w295) -> ("error out"=w300:errorcluster, "instrument handle out"=w297:refnum<k15>)  [unwired: 7 in]
                n96 = call <instrlib>:"niDCPower Initiate With Channels.vi"("error in (no error)"=w300, "channel name"=w293, "instrument handle"=w294) -> ("error out"=w298:errorcluster, "instrument handle out"=w299:refnum<k15>)  [unwired: 7 in]
              }
              frame #1 {
                w307 = T5 1033 items=["Source Complete Event"=1030, "Measure Complete Event"=1031, "Sequence Iteration Complete Event"=1032, "Sequence Engine Done Event"=1033] ("event")
                n97 = call <instrlib>:"niDCPower Wait For Event With Channels.vi"("timeout (10.0)"=w301, "error in (no error)"=w306, "event"=w307, "channel name"=w302, "instrument handle"=w303) -> ("error out"=w304:errorcluster, "instrument handle out"=w305:refnum<k15>)  [unwired: 5 in]
              }
            }
            n98 = Bundle By Name(cluster=w281, "Source out"=w280, "Load out"=w279) -> (w278:T3)
          }
          frame "PerformMeasurement" {
            # "1.Fetches the voltages and currents of both the PPS and E-Load\n2.Calculates the efficiency (%), load voltage deviation (%)"
            n99 = Unbundle By Name(w316) -> ("Nominal output voltage"=w312:dbl)
            n100 = call "Perform Measurements.vi"("error in"=w318, "Measurement Context"=w310, "Nominal output voltage"=w312, "Reference values"=w311) -> ("error out"=w317:errorcluster, "Measurement Results"=w313:T1, "Load out"=w314:refnum<k15>, "Source out"=w315:refnum<k15>)  [unwired: 3 in]
            n101 = Bundle By Name(cluster=w311, "Source out"=w315, "Load out"=w314, "Measurement Results"=w313) -> (w309:T3)
          }
          frame "Exit", Default {
            # "1. Aborts the channels\n2. Deletes the created advanced sequence\n3. Close all the opened sessions"
            n102 = Release Queue(queue=w320, error in (no error)=w325) -> (error out=w324:errorcluster)  [unwired: 1 in, 2 out]
            n103 = case shown="No Error" w324 {
              selector: w324 -> [w327 w358]
              tunnel: [w326 w357] -> w322
              tunnel: w323 -> [w328 w356]
              tunnel: [w341 w356] -> w321
              frame No Error {
                # "Updates the status indicator on the operation performed if there is no error"
                n104 = Unbundle By Name(w328) -> ("Source out"=w339:refnum<k15>, "Source channel name"=w333:string, "Source sequence name"=w329:string, "Load out"=w338:refnum<k15>, "Load channel name"=w337:string)
                n105 = call <instrlib>:"niDCPower Abort With Channels.vi"("error in (no error)"=w327, "channel name"=w337, "instrument handle"=w338) -> ("error out"=w340:errorcluster, "instrument handle out"=w330:refnum<k15>)  [unwired: 7 in]
                n106 = call <instrlib>:"niDCPower Close.vi"("error in (no error)"=w340, "instrument handle"=w330) -> ("error out"=w332:errorcluster)  [unwired: 9 in]
                n107 = call <instrlib>:"niDCPower Abort With Channels.vi"("error in (no error)"=w332, "channel name"=w333, "instrument handle"=w339) -> ("error out"=w335:errorcluster, "instrument handle out"=w334:refnum<k15>)  [unwired: 7 in]
                n108 = call <instrlib>:"niDCPower Delete Advanced Sequence With Channels.vi"("error in (no error)"=w335, "sequence name"=w329, "channel name"=w333, "instrument handle"=w334) -> ("error out"=w336:errorcluster, "instrument handle out"=w331:refnum<k15>)  [unwired: 6 in]
                n109 = call <instrlib>:"niDCPower Close.vi"("error in (no error)"=w336, "instrument handle"=w331) -> ("error out"=w326:errorcluster)  [unwired: 9 in]
                n110 = Bundle By Name(cluster=w328, "Measurement Results.Status"="The measurement is performed successfully" ("message")) -> (w341:T3)
              }
              frame Error {
                # "Resets the device with default values whenever there is an error"
                n111 = Unbundle By Name(w356) -> ("Source out"=w347:refnum<k15>, "Source channel name"=w345:string, "Load out"=w344:refnum<k15>, "Load channel name"=w343:string)
                n112 = call <instrlib>:"niDCPower Abort With Channels.vi"("error in (no error)"=w358, "channel name"=w343, "instrument handle"=w344) -> ("error out"=w351:errorcluster, "instrument handle out"=w348:refnum<k15>)  [unwired: 7 in]
                n113 = call <instrlib>:"niDCPower Reset With Channels.vi"("error in (no error)"=w351, "channel name"=w343, "instrument handle"=w348) -> ("error out"=w352:errorcluster, "instrument handle out"=w353:refnum<k15>)  [unwired: 7 in]
                n114 = call <instrlib>:"niDCPower Close.vi"("error in (no error)"=w352, "instrument handle"=w353) -> ("error out"=w346:errorcluster)  [unwired: 9 out]
                n115 = call <instrlib>:"niDCPower Abort With Channels.vi"("error in (no error)"=w346, "channel name"=w345, "instrument handle"=w347) -> ("error out"=w349:errorcluster, "instrument handle out"=w350:refnum<k15>)  [unwired: 7 in]
                n116 = call <instrlib>:"niDCPower Reset With Channels.vi"("error in (no error)"=w349, "channel name"=w345, "instrument handle"=w350) -> ("error out"=w355:errorcluster, "instrument handle out"=w354:refnum<k15>)  [unwired: 7 in]
                n117 = call <instrlib>:"niDCPower Close.vi"("error in (no error)"=w355, "instrument handle"=w354) -> ("error out"=w357:errorcluster)  [unwired: 9 out]
              }
            }
          }
        }
      }
    }
    frame "Power off the DUT" {
      # "Stops generation on the output channel and resets the channels to default values"
      n118 = Unbundle By Name(w377) -> ("Source resource name"=w379:string, "Load resource name"=w382:string)
      n119 = call <instrlib>:"niDCPower Initialize With Independent Channels.vi"("error in (no error)"=w389, "resource name"=w382) -> ("error out"=w383:errorcluster, "instrument handle out"=w381:refnum<k15>)  [unwired: 8 in]
      n120 = call-poly <instrlib>:"niDCPower Get Channel Name (Poly).vi"("error in (no error)"=w383, "index"="0", "instrument handle"=w381) -> ("error out"=w394:errorcluster, "name"=w391:string, "instrument handle out"=w392:refnum<k15>)  [unwired: 6 in]
      n121 = call <instrlib>:"niDCPower Configure Output Enabled.vi"("error in (no error)"=w394, "output enabled"=FALSE, "channel name"=w391, "instrument handle"=w392) -> ("error out"=w401:errorcluster, "instrument handle out"=w400:refnum<k15>)  [unwired: 6 in]
      n122 = call <instrlib>:"niDCPower Reset With Channels.vi"("error in (no error)"=w401, "channel name"=w391, "instrument handle"=w400) -> ("error out"=w395:errorcluster, "instrument handle out"=w396:refnum<k15>)  [unwired: 7 in]
      n123 = call <instrlib>:"niDCPower Close.vi"("error in (no error)"=w395, "instrument handle"=w396) -> ("error out"=w386:errorcluster)  [unwired: 9 out]
      n124 = call <instrlib>:"niDCPower Initialize With Independent Channels.vi"("error in (no error)"=w386, "resource name"=w379) -> ("error out"=w380:errorcluster, "instrument handle out"=w378:refnum<k15>)  [unwired: 8 in]
      n125 = call-poly <instrlib>:"niDCPower Get Channel Name (Poly).vi"("error in (no error)"=w380, "index"="0", "instrument handle"=w378) -> ("error out"=w385:errorcluster, "name"=w384:string, "instrument handle out"=w387:refnum<k15>)  [unwired: 6 in]
      n126 = call <instrlib>:"niDCPower Reset With Channels.vi"("error in (no error)"=w385, "channel name"=w384, "instrument handle"=w387) -> ("error out"=w398:errorcluster, "instrument handle out"=w397:refnum<k15>)  [unwired: 7 in]
      n127 = call <instrlib>:"niDCPower Close.vi"("error in (no error)"=w398, "instrument handle"=w397) -> ("error out"=w390:errorcluster)  [unwired: 9 out]
      n128 = Bundle By Name(cluster=w375, "Measurement Results.Status"="The DUT is powered OFF") -> (w373:T3)
    }
  }
  "error out" <- w1
  "measure call context out" <- w3
  n129 = Unbundle By Name(w2) -> ("Measurement Results"=→"measurement results":T1)
